vi "Watchdog Open.vi"(4 "error in (no error)":errorcluster, 7 "disable watchdog on VI exit (T)":bool=TRUE) -> (0 "error out":errorcluster, 3 "watchdogID":u64 format="%.0x")   [LabVIEW 2025]
doc: "<p>Opens a watchdog session using the first available <a href=\"nihelplauncher://docs/csh?context=lvrt_lvrtconcepts_rt_watchdog\">watchdog object</a>.</p>"
uses:
  niwd4c.dll
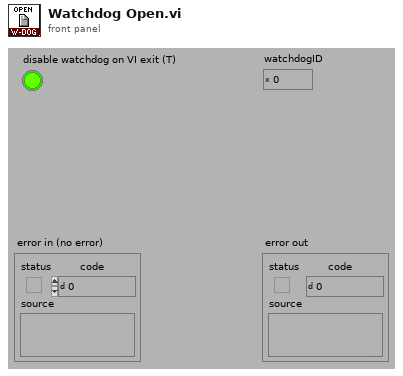
[diagram p1: front panel]
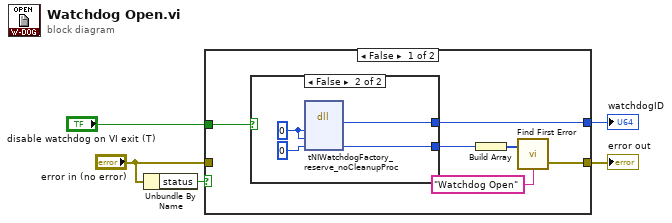
[diagram p0: block diagram]
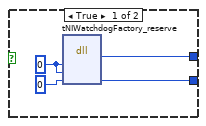
[diagram p2: hidden frame]
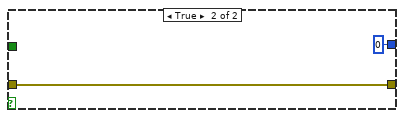
[diagram p3: hidden frame]
diagram:
  n1 = Unbundle By Name("error in (no error)") -> ("status"=w3:bool)
  n2 = case shown="False" w3 {
    tunnel: [w8 u32 0] -> w5
    tunnel: [w10 w21] -> w4
    tunnel: "error in (no error)" -> [_ w21]
    tunnel: "disable watchdog on VI exit (T)" -> [w6 _]
    frame False {
      n3 = case shown="False" w6 {
        tunnel: [w15 w19] -> w8
        tunnel: [w14 w18] -> w7
        frame True {
          w13 = u32 0 ("identifier")
          n4 = dll-call lib="niwd4c.*" fn="tNIWatchdogFactory_reserve" label="Reserve"("identifier"=w13, "instance"=w13, "status"=0 ("identifier")) -> ("return type"=w15:u64, "status"=w14:i32)  [unwired: 5 in, 2 out]
        }
        frame False {
          w17 = u32 0 ("identifier")
          n5 = dll-call lib="niwd4c.*" fn="tNIWatchdogFactory_reserve_noCleanupProc" label="Reserve_noCleanupProc"("identifier"=w17, "instance"=w17, "status"=0 ("identifier")) -> ("return type"=w19:u64, "status"=w18:i32)  [unwired: 5 in, 2 out]
        }
      }
      n6 = Build Array(w7) -> (w11:i32[])
      n7 = call <vilib>:"Find First Error.vi"("source messages"="Watchdog Open", "error codes"=w11) -> ("error out"=w10:errorcluster)  [unwired: 2 in, 1 out]
    }
    frame True {
    }
  }
  "error out" <- w4
  "watchdogID" <- w5
